vi "RemoteVI Status Panel.vi"(0 "stop":bool) -> ()   [LabVIEW 2020, in "RemoteVI.lvlib"]
doc: "A small window that shows what RemoteVI shares in this LabVIEW application instance (the text of RemoteVI Status.vi: per share its link, target, clients, frame rate, data rate and last error), refreshed every 500 ms. RemoteVI Show Status.vi opens it; you can also run it yourself, or insert it into a subpanel of your own UI (Insert VI, then Run VI without waiting). It ends when its window is closed, on Close, or when stop is set TRUE (Control Value.Set by name - the way to end it in a subpanel). It only reads the status; closing it stops no share."
uses:
  RemoteVI.lvlib
panel:
  out "Shares":string
  in  "Close":bool
  in  "tick":bool
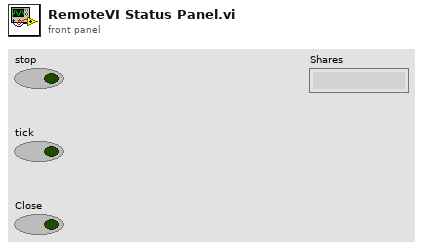
[diagram p1: front panel]
types:
  T1 = cluster{"label":string, "left":i32, "top":i32, "width":i32, "height":i32}[]
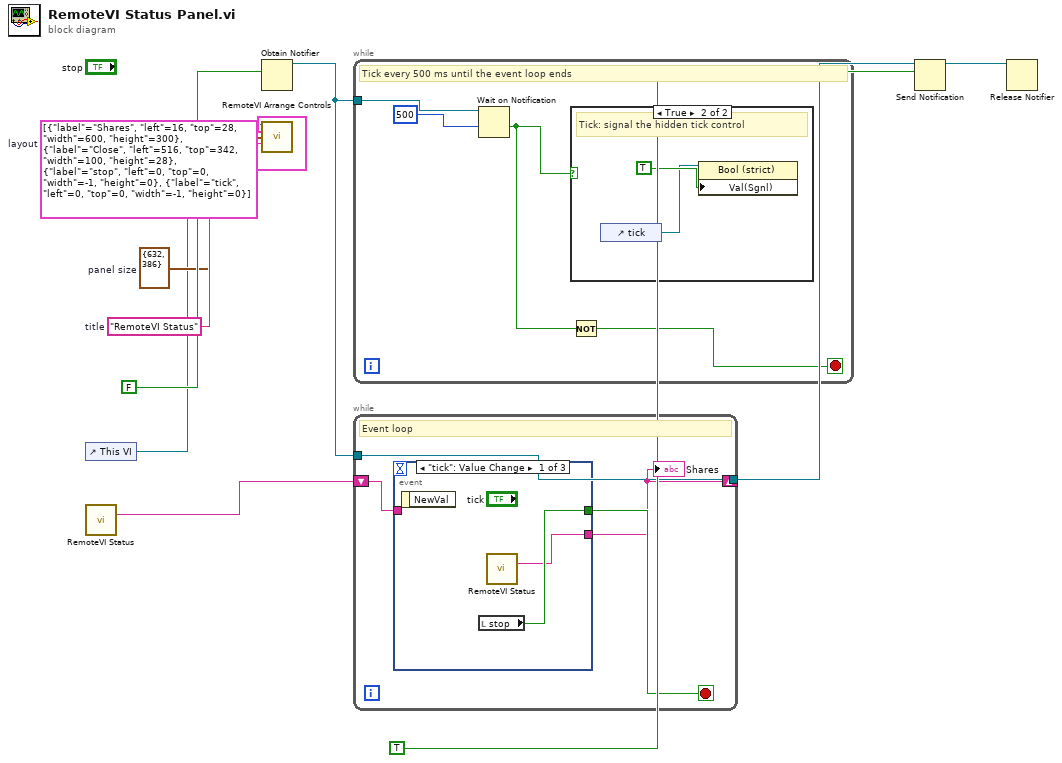
[diagram p0: block diagram]
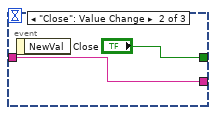
[diagram p2: hidden frame]
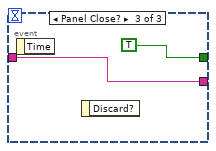
[diagram p3: hidden frame]
diagram:
  w4 = "RemoteVI Status"  # title
  w3 = cluster{"width":i32, "height":i32} {"width"=632, "height"=386}  # panel size
  w2 = T1 [{"label"="Shares", "left"=16, "top"=28, "width"=600, "height"=300}, {"label"="Close", "left"=516, "top"=342, "width"=100, "height"=28}, {"label"="stop", "left"=0, "top"=0, "width"=-1, "height"=0}, {"label"="tick", "left"=0, "top"=0, "width"=-1, "height"=0}]  # layout
  n1 = control-ref of="This VI"() -> (w1:refnum<vi>)
  n2 = call "RemoteVI Status.vi"() -> ("text"=w5:string)  [unwired: 14 in, 1 out]
  n3 = Obtain Notifier(notification data type=FALSE) -> (notifier out=w7:refnum<notifier>)  [unwired: 3 in, 2 out]
  n4 = call "RemoteVI Arrange Controls.vi"("VI"=w1, "layout"=w2, "panel size"=w3, "title"=w4) -> ()  [unwired: 12 in]
  n5 = while {
    tunnel: w7 -> [w11]
    stop <- w14 stop-if-true
    # "Tick every 500 ms until the event loop ends"
    n6 = Wait on Notification(notifier=w11, timeout in ms (-1)=500) -> (timed out?=w13:bool)  [unwired: 2 in, 3 out]
    n7 = case shown="True" w13 {
      frame False {
      }
      frame True {
        # "Tick: signal the hidden tick control"
        n8 = control-ref of="tick"() -> (w15:refnum<vi>)
        n9 = property class="Bool (strict)"(reference=w15, "Val(Sgnl)"=TRUE) -> ()  [unwired: 1 in, 2 out]
      }
    }
    n10 = Not(x=w13) -> (.not. x?=w14:bool)
  }
  n11 = while {
    tunnel: w7 -> [w17]
    shift-right: [w19] -> _
    shift-left: w5 -> [w18]
    tunnel: [w17] -> w8
    stop <- w20 stop-if-true
    # "Event loop"
    n12 = event shown="[0] \"tick\": Value Change" {
      selector: _ -> [_ _ _]
      dyn-events: _ -> [_ _ _]
      timeout: _ -> [_ _ _]
      tunnel: [w22 "Close" TRUE] -> w20
      tunnel: [w21 w23 w25] -> w19
      tunnel: w18 -> [_ w23 w25]
      event "tick": Value Change {
        n13 = event-data() -> ()  [unwired: 1 in, 1 out]
        n14 = local read "stop"() -> (w22:bool)
        n15 = call "RemoteVI Status.vi"() -> ("text"=w21:string)  [unwired: 14 in, 1 out]
      }
      event "Close": Value Change {
        n16 = event-data() -> ()  [unwired: 1 in, 1 out]
      }
      event Panel Close? {
        n17 = event-data() -> ()  [unwired: 1 in, 1 out]
        n18 = event-data() -> ()  [unwired: 2 in, 1 out]
      }
    }
    "Shares" <- w19
  }
  n19 = Send Notification(notification=TRUE, notifier=w8) -> (notifier out=w10:refnum<notifier>)  [unwired: 1 in, 1 out]
  n20 = Release Notifier(notifier=w10) -> ()  [unwired: 2 in, 3 out]
